vi "CarayaCLIExecutionEngine.vi"() -> ()   [LabVIEW 2020]
uses:
  <vilib>/addons/_JKI Toolkits/Caraya/run-tests/Run Test (Scalar Path).vi
  <vilib>/Wiresmith Technology/G CLI/CLI Class/CLI.lvclass
  <vilib>/addons/_JKI Toolkits/Caraya/Caraya.lvlib
panel:
  out "exit LabVIEW":bool
  out "error out":errorcluster
  out "Application:Command Line Arguments":string[](array[string])
  out "recursive":bool
  out "verbose":bool
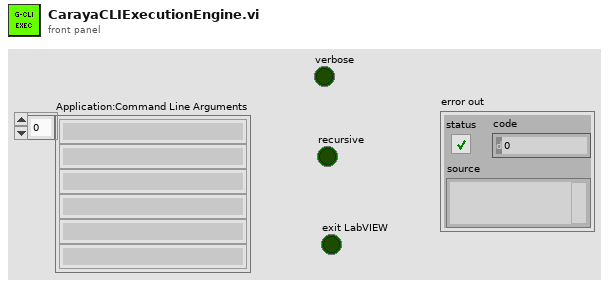
[diagram p1: front panel]
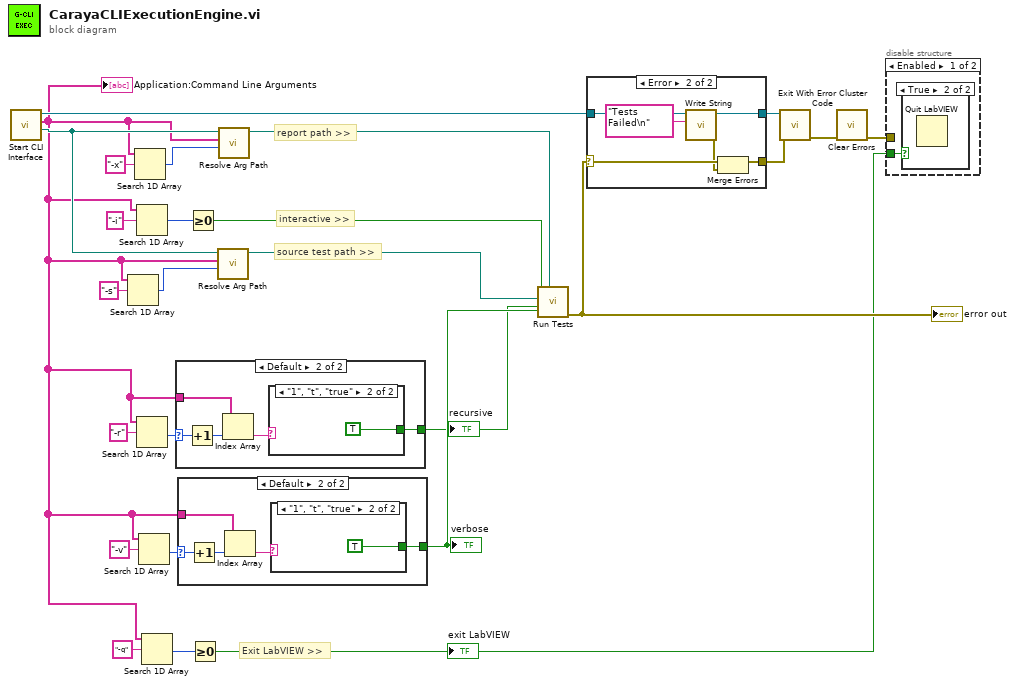
[diagram p0: block diagram]
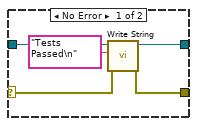
[diagram p4: hidden frame]
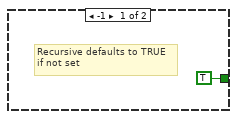
[diagram p5: hidden frame]
diagram:
  # "Exit LabVIEW >>"
  # "source test path >>"
  # "interactive >>"
  # "report path >>"
  n1 = call <vilib>:"Start CLI Interface.vi"() -> ("Working Directory"=w4:path, "Custom Parameters"=w3:string[], "CLI out"=w16:refnum<class "CLI.lvclass">)  [unwired: 8 in, 1 out]
  "Application:Command Line Arguments" <- w3
  n2 = Search 1D Array(1D array=w3, element="-s") -> (index of element=w2:i32)  [unwired: 1 in]
  n3 = Search 1D Array(1D array=w3, element="-x") -> (index of element=w19:i32)  [unwired: 1 in]
  n4 = Search 1D Array(1D array=w3, element="-i") -> (index of element=w25:i32)  [unwired: 1 in]
  n5 = Search 1D Array(1D array=w3, element="-r") -> (index of element=w22:i32)  [unwired: 1 in]
  n6 = Search 1D Array(1D array=w3, element="-v") -> (index of element=w23:i32)  [unwired: 1 in]
  n7 = Search 1D Array(1D array=w3, element="-q") -> (index of element=w6:i32)  [unwired: 1 in]
  n8 = case shown="Default" w22 {
    selector: w22 -> [_ w29]
    tunnel: [TRUE w30] -> w12
    tunnel: w3 -> [_ w28]
    frame -1 {
      # "Recursive defaults to TRUE\nif not set"
    }
    frame Default {
      n9 = Increment(x=w29) -> (x+1=w32:i32)
      n10 = Index Array(array=w28, index=w32) -> (element=w31:string)
      n11 = case shown="\"1\", \"t\", \"true\"" w31 {
        tunnel: [_ TRUE] -> w30
        frame Default {
        }
        frame "1", "t", "true" {
        }
      }
    }
  }
  "recursive" <- w12
  n12 = case shown="Default" w23 {
    selector: w23 -> [_ w35]
    tunnel: [_ w36] -> w17
    tunnel: w3 -> [_ w34]
    frame -1 {
      # "Verbosity defaults to False\nif not set"
    }
    frame Default {
      n13 = Increment(x=w35) -> (x+1=w38:i32)
      n14 = Index Array(array=w34, index=w38) -> (element=w37:string)
      n15 = case shown="\"1\", \"t\", \"true\"" w37 {
        tunnel: [_ TRUE] -> w36
        frame Default {
        }
        frame "1", "t", "true" {
        }
      }
    }
  }
  "verbose" <- w17
  n16 = Greater Or Equal To 0?(x=w25) -> (x >= 0?=w13:bool)
  n17 = Greater Or Equal To 0?(x=w6) -> (x >= 0?=w5:bool)
  "exit LabVIEW" <- w5
  n18 = call "Resolve Arg Path.vi"("index of element"=w2, "Custom Parameters"=w3, "Working Directory"=w4) -> ("Resolved Path"=w1:path)  [unwired: 8 in]
  n19 = call "Resolve Arg Path.vi"("index of element"=w19, "Custom Parameters"=w3, "Working Directory"=w4) -> ("Resolved Path"=w14:path)  [unwired: 8 in]
  n20 = call-poly <vilib>:"Run Tests.vi"("Verbose"=w17, "Report Path"=w14, "Inspect Recursively (T)"=w12, "Test Path"=w1, "Interactive (T)"=w13) -> ("error out"=w15:errorcluster)  [unwired: 5 in, 1 out]
  "error out" <- w15
  n21 = case shown="Error" w15 {
    selector: w15 -> [w41 w47]
    tunnel: w16 -> [w44 w50]
    tunnel: [w43 w49] -> w10
    tunnel: [w40 w45] -> w9
    frame No Error {
      n22 = call <vilib>:"Write String.vi"("error in (no error)"=w41, "Text to Write"="Tests Passed\n", "CLI in"=w44) -> ("error out"=w40:errorcluster, "CLI out"=w43:refnum<class "CLI.lvclass">)  [unwired: 7 in]
    }
    frame Error {
      n23 = call <vilib>:"Write String.vi"("Text to Write"="Tests Failed\n", "CLI in"=w50) -> ("error out"=w46:errorcluster, "CLI out"=w49:refnum<class "CLI.lvclass">)  [unwired: 8 in]
      n24 = Merge Errors(w47, w46) -> (w45:errorcluster)
    }
  }
  n25 = call <vilib>:"Exit With Error Cluster Code.vi"("error in (no error)"=w9, "CLI in"=w10) -> ("error out"=w11:errorcluster)  [unwired: 9 in]
  n26 = call <vilib>:"Clear Errors.vi"("error in (no error)"=w11) -> ("error out"=w8:errorcluster)  [unwired: 5 in, 1 out]
  n27 = disable-structure shown="Enabled" {
    disable-tunnel: w8 -> [_ _]
    disable-tunnel: w5 -> [w51 _]
    frame Enabled {
      n28 = case shown="True" w51 {
        frame False {
        }
        frame True {
          n29 = Quit LabVIEW() -> ()  [unwired: 1 in]
        }
      }
    }
    frame Disabled {
    }
  }
